vi "Set Live img window UI from file-Boolean.vi"(8 "error in (no error)":errorcluster, 9 "Keys setup.Boolean":T2, 10 "Section name":string, 11 "Refnum in":T1) -> (0 "error out":errorcluster, 3 "Refnum out":T1)   [LabVIEW 2020]
uses:
  Typedefs/Ini file interface (Boolean).ctl
  <vilib>/Utility/config.llb/Config Data RefNum.ctl
  User Interface/Globals/gl_Windows Ctrl refs.vi
  <vilib>/Utility/config.llb/NI_LVConfig.lvlib
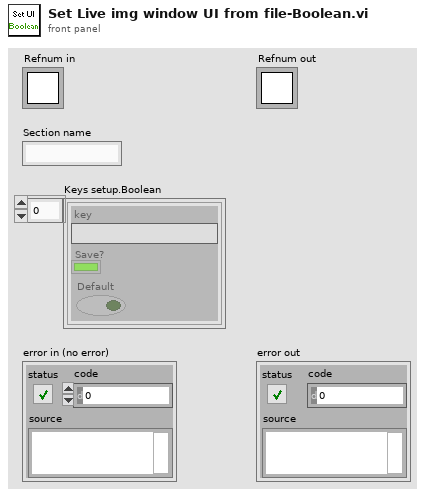
[diagram p1: front panel]
types:
  T1 = typedef "NI_LVConfig.lvlib/Config Data RefNum.ctl" = refnum<k1>
  T2 = typedef "Ini file interface (Boolean).ctl" = cluster{"key":string, "Save?":bool, "Default":bool}[]
  T3 = typedef "Live window-ctrl refs.ctl" = cluster{"This VI":refnum<vi>, "Pane":refnum<vi>, "Show REF Image Left":refnum<vi>, "Show REF Image Right":refnum<vi>, "Snapshot":refnum<vi>, "Left Image Palette":refnum<vi>, "Right Image Palette":refnum<vi>, "Left Channel":refnum<vi>, "Right Channel":refnum<vi>, "Left image intensity":refnum<vi>, "Right image intensity":refnum<vi>, "Left Image Display":T4, "Right Image Display":T4, "Refresh rate ind (Hz)":refnum<vi>, "Acq rate ind (Hz)":refnum<vi>, "Stop (ind)":refnum<vi>}
  T4 = typedef "Image display ref.ctl" = refnum<vi>
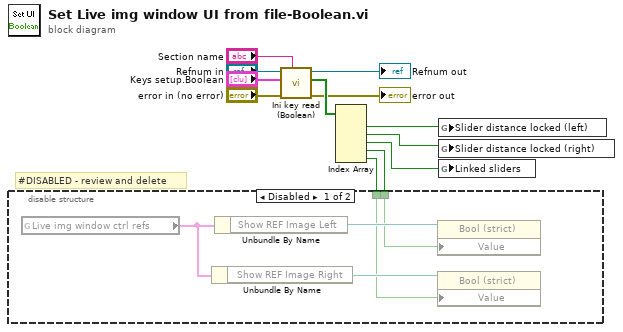
[diagram p0: block diagram]
diagram:
  # "#DISABLED - review and delete"
  n1 = call "Ini key read (Boolean).vi"("Section"="Section name", "error in (no error)"="error in (no error)", "Parameter names & setup"="Keys setup.Boolean", "Ini file refnum in"="Refnum in") -> ("error out"=→"error out":errorcluster, "Value read/used"=w12:bool[], "Ini file refnum out"=→"Refnum out":T1)  [unwired: 5 in]
  n2 = Index Array(array=w12) -> (element #1=w5:bool, element #2=w4:bool, element #3=w3:bool, element #4=w2:bool, element #5=w1:bool)  [unwired: 5 in]
  n3 = disable-structure shown="Disabled" {
    disable-tunnel: w2 -> [w14 _]
    disable-tunnel: w1 -> [w13 _]
    frame Disabled {
      n4 = global read "gl_Windows Ctrl refs.vi" "Live img window ctrl refs"() -> (w15:T3)
      n5 = Unbundle By Name(w15) -> ("Show REF Image Right"=w16:refnum<vi>)
      n6 = Unbundle By Name(w15) -> ("Show REF Image Left"=w17:refnum<vi>)
      n7 = property class="Bool (strict)"(reference=w17, "Value"=w14) -> ()  [unwired: 1 in, 2 out]
      n8 = property class="Bool (strict)"(reference=w16, "Value"=w13) -> ()  [unwired: 1 in, 2 out]
    }
    frame Enabled {
    }
  }
  n9 = global write "gl_Windows Ctrl refs.vi" "Slider distance locked (left)"(w5) -> ()
  n10 = global write "gl_Windows Ctrl refs.vi" "Slider distance locked (right)"(w4) -> ()
  n11 = global write "gl_Windows Ctrl refs.vi" "Linked sliders"(w3) -> ()
